vi "Read String Input.vi"(8 "error in (no error)":errorcluster, 10 "String Input in":T1, 11 "Modbus in":refnum<class "Modbus.lvclass">) -> (0 "error out":errorcluster, 2 "String Value":string, 3 "Modbus out":refnum<class "Modbus.lvclass">)   [LabVIEW 2026, in "Modbus.lvlib" / "Modbus.lvclass"]
uses:
  Modbus.lvclass
  Types/String Data.ctl
  Types/Modbus Table.ctl
  Modbus.lvclass/Modbus.ctl
  <vilib>/ni/Modbus Library/API/Master/Modbus Master.lvclass
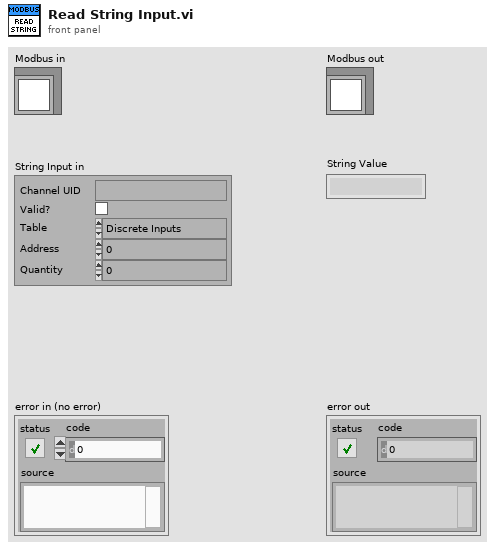
[diagram p1: front panel]
types:
  T1 = typedef "Modbus.lvlib/Modbus.lvclass/String Data.ctl" = cluster{"Channel UID":string, "Valid?":bool, "Table":T2, "Address":i32, "Quantity":u16}
  T2 = typedef "Modbus.lvlib/Modbus.lvclass/Modbus Table.ctl" = enum16{"Discrete Inputs", "Coils", "Input Registers", "Holding Registers"}
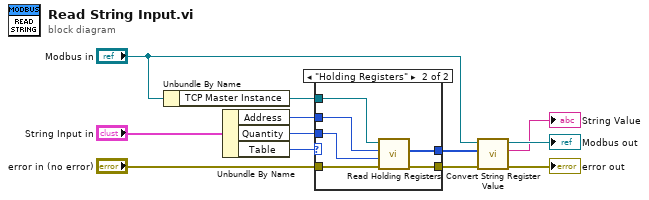
[diagram p0: block diagram]
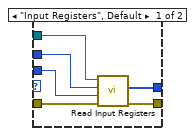
[diagram p2: hidden frame]
diagram:
  n1 = Unbundle By Name("Modbus in") -> ("TCP Master Instance"=w10:refnum<class "Modbus Master.lvclass">)
  n2 = Unbundle By Name("String Input in") -> ("Address"=w9:i32, "Quantity"=w8:u16, "Table"=w7:T2)
  n3 = case shown="\"Holding Registers\"" w7 {
    tunnel: w10 -> [w18 w24]
    tunnel: [w17 w23] -> w5
    tunnel: w9 -> [w16 w22]
    tunnel: [w15 w21] -> w2
    tunnel: w8 -> [w14 w20]
    tunnel: "error in (no error)" -> [w13 w19]
    frame "Input Registers", Default {
      n4 = call-dynamic "Read Input Registers.vi"("error in"=w13, "number of inputs"=w14, "starting address"=w16, "Modbus master in"=w18) -> ("error out"=w17:errorcluster, "register values"=w15:u16[])  [unwired: 5 in, 1 out]
    }
    frame "Holding Registers" {
      n5 = call-dynamic "Read Holding Registers.vi"("error in"=w19, "number of inputs"=w20, "starting address"=w22, "Modbus master in"=w24) -> ("error out"=w23:errorcluster, "register values"=w21:u16[])  [unwired: 5 in, 1 out]
    }
  }
  n6 = call "Convert String Register Value.vi"("error in (no error)"=w5, "Register Values"=w2, "Modbus in"="Modbus in") -> ("error out"=→"error out":errorcluster, "String out"=→"String Value":string, "Modbus out"=→"Modbus out":refnum<class "Modbus.lvclass">)  [unwired: 6 in]
